vi "[ce] ODE Solver - Prepare variables.vi"(4 "method":enum16{"Runge Kutta", "Euler"}(ring), 6 "equation parameters":T1(array[cluster]) {"x0" format="%.2f"}, 7 "VC Handle":T4, 8 "error in":errorcluster, 9 "h value":dbl format="%.5f", 10 "time value":dbl format="%.2f", 11 "time":string="t") -> (0 "error out":errorcluster, 1 "variable names":T2(array[cluster]), 2 "time names":T3, 5 "dup VC Handle":T4)   [LabVIEW 2021]
doc: "::: CalcExpress Toolkit :::\nCopyright (c) 2000-2026 Konstantin Shifershteyn. All rights reserved."
uses:
  cetypes.llb/VarMan Variable Context Handle.ctl
panel:
  # "="
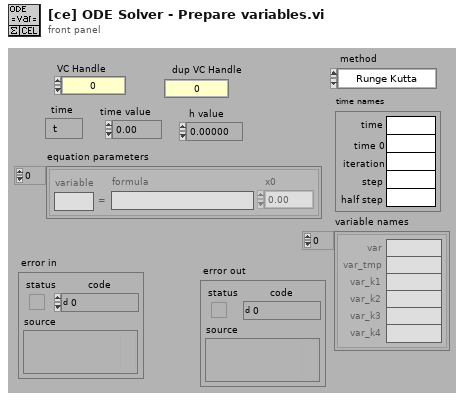
[diagram p1: front panel]
types:
  T1 = cluster{"variable":string, "formula":string, "x0":dbl}[]
  T2 = cluster{"var":string, "var_tmp":string, "var_k1":string, "var_k2":string, "var_k3":string, "var_k4":string}[]
  T3 = cluster{"time":string, "time 0":string, "iteration":string, "step":string, "half step":string}
  T4 = typedef "VarMan Variable Context Handle.ctl" = i32
  T5 = enum16{"create", "destroy", "set value", "get value"}
  T6 = typedef "VarMan Error Code.ctl" = u16
  T7 = cluster{"[0]":string, "[1]":string, "[2]":string, "[3]":string, "[4]":string, "[5]":string}
  T8 = cluster{"[0]":string, "[1]":string, "[2]":string, "[3]":string, "[4]":string}
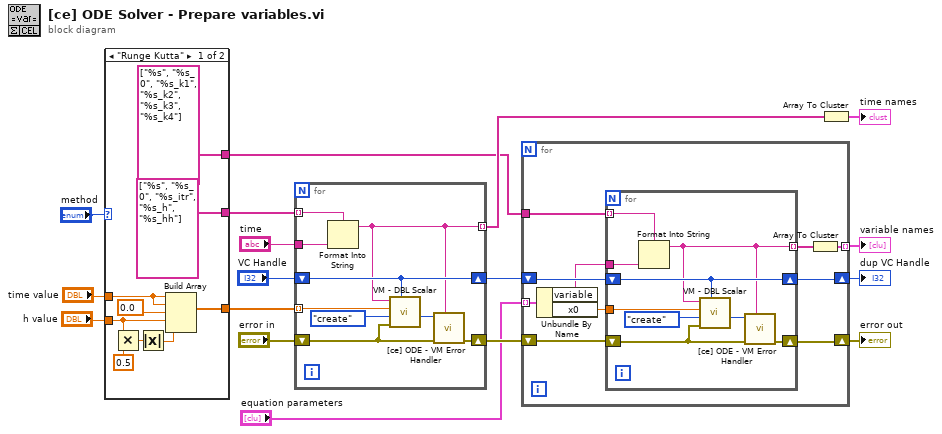
[diagram p0: block diagram]
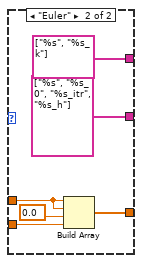
[diagram p2: hidden frame]
diagram:
  n1 = case shown="\"Runge Kutta\"" "method" {
    tunnel: "time value" -> [w21 w29]
    tunnel: "h value" -> [w20 w27]
    tunnel: [string[] ["%s", "%s_0", "%s_itr", "%s_h", "%s_hh"] string[] ["%s", "%s_0", "%s_itr", "%s_h"]] -> w4
    tunnel: [w25 w32] -> w5
    tunnel: [string[] ["%s", "%s_0", "%s_k1", "%s_k2", "%s_k3", "%s_k4"] string[] ["%s", "%s_k"]] -> w7
    frame "Runge Kutta" {
      n2 = Multiply(x=w20, y=0.5) -> (x*y=w19:dbl)
      n3 = Absolute Value(x=w19) -> (abs(x)=w18:dbl)
      n4 = Build Array(w21, w21, 0.0, w20, w18) -> (w25:dbl[])
    }
    frame "Euler" {
      n5 = Build Array(w29, w29, 0.0 ("Input Element"), w27) -> (w32:dbl[])
    }
  }
  n6 = for {
    shift-right: [w38] -> w10
    shift-left: "error in" -> [w33]
    shift-right: [w40] -> w11
    shift-left: "VC Handle" -> [w40]
    tunnel: w4 -> [w37] mode=indexing
    tunnel: w5 -> [w36] mode=indexing
    tunnel: "time" -> [w35]
    tunnel: [w34] -> w15 mode=indexing
    n7 = Format Into String(format string=w37, w35) -> (resulting string=w34:string)  [unwired: 2 in, 1 out]
    n8 = call "VM - DBL Scalar.vi"("VC Handle"=w40, "error in"=w33, "cmd"=T5."create", "value in"=w36, "name_spec"=w34) -> ("err code"=w39:T6)  [unwired: 1 in, 5 out]
    n9 = call "[ce] ODE - VM Error Handler.vi"("var name"=w34, "error before"=w33, "err code"=w39) -> ("error out"=w38:errorcluster)  [unwired: 6 in]
  }
  n10 = for {
    shift-right: [w50] -> w3
    shift-left: w11 -> [w48]
    tunnel: [w49] -> w12 mode=indexing
    shift-right: [w46] -> w9
    shift-left: w10 -> [w47]
    tunnel: w7 -> [w45]
    tunnel: "equation parameters" -> [w42] mode=indexing
    n11 = Unbundle By Name(w42) -> ("variable"=w43:string, "x0"=w44:dbl)
    n12 = for {
      shift-right: [w57] -> w46
      shift-left: w47 -> [w52]
      shift-right: [w59] -> w50
      shift-left: w48 -> [w59]
      tunnel: w45 -> [w56] mode=indexing
      tunnel: w44 -> [w55]
      tunnel: [w54] -> w51 mode=indexing
      tunnel: w43 -> [w53]
      n13 = Format Into String(format string=w56, w53) -> (resulting string=w54:string)  [unwired: 2 in, 1 out]
      n14 = call "VM - DBL Scalar.vi"("VC Handle"=w59, "error in"=w52, "cmd"=T5."create", "value in"=w55, "name_spec"=w54) -> ("err code"=w58:T6)  [unwired: 1 in, 5 out]
      n15 = call "[ce] ODE - VM Error Handler.vi"("var name"=w54, "error before"=w52, "err code"=w58) -> ("error out"=w57:errorcluster)  [unwired: 6 in]
    }
    n16 = Array To Cluster(array=w51) -> (cluster=w49:T7)
  }
  "error out" <- w9
  "dup VC Handle" <- w3
  "variable names" <- w12
  n17 = Array To Cluster(array=w15) -> (cluster=→"time names":T8)
